vi "Get String Channel Name.vi"(9 "Channel Numer":i32) -> (1 "Bool Channel Name":string, 2 "Bool Channel ID":string)   [LabVIEW 2026, in "Modbus.lvlib" / "Modbus.lvclass"]
uses:
  Modbus.lvclass
  Globals/Modbus Strings.vi
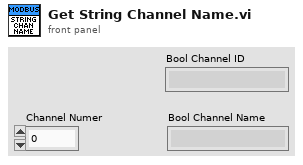
[diagram p1: front panel]
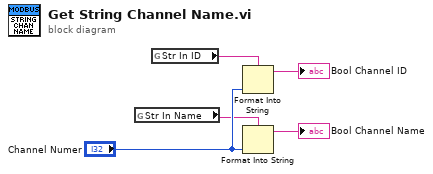
[diagram p0: block diagram]
diagram:
  n1 = global read "Modbus Strings.vi" "Str In Name"() -> (w1:string)
  n2 = global read "Modbus Strings.vi" "Str In ID"() -> (w2:string)
  n3 = Format Into String(format string=w2, "Channel Numer") -> (resulting string=→"Bool Channel ID":string)  [unwired: 2 in, 1 out]
  n4 = Format Into String(format string=w1, "Channel Numer") -> (resulting string=→"Bool Channel Name":string)  [unwired: 2 in, 1 out]
